vi "Sorted ARR Data.vi"(10 "Uart-num":string[](array[string])=["11", "15"], 11 "Data":string[][](array[string])=[["0", "11", "12"], ["15", "11", "11"], ["11", "11", "11"], ["12", "11", "11"], ["15", "11", "11"]]) -> (2 "Consistent":bool, 3 "Data-Sorted":string[][](array[string]))   [LabVIEW 2025, in "G-Uart-Class.lvclass"]
uses:
  G-Uart-Class.lvclass
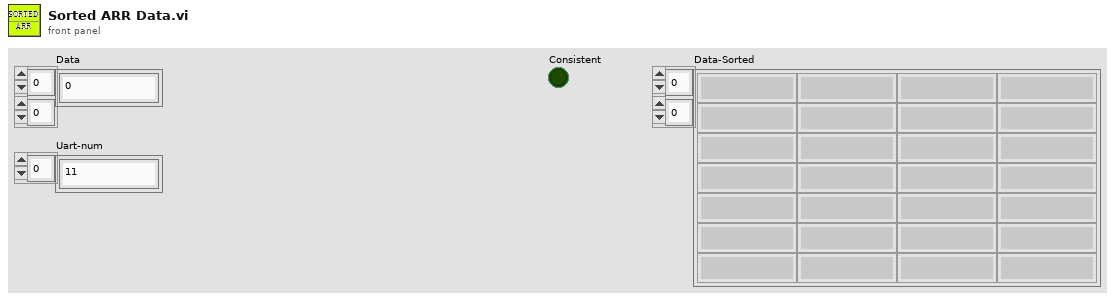
[diagram p1: front panel]
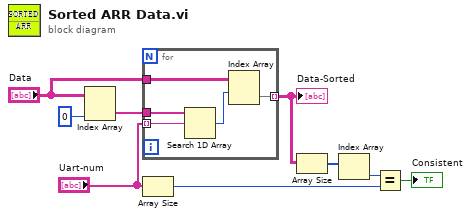
[diagram p0: block diagram]
diagram:
  n1 = Index Array(array="Data", index (col)=0 ("禁用的索引 (列)")) -> (element=w8:string[])  [unwired: 1 in]
  n2 = for {
    tunnel: w8 -> [w13]
    tunnel: "Uart-num" -> [w14] mode=indexing
    tunnel: "Data" -> [w12]
    tunnel: [w10] -> w1 mode=indexing
    n3 = Search 1D Array(1D array=w13, element=w14) -> (index of element=w11:i32)  [unwired: 1 in]
    n4 = Index Array(array=w12, index (row)=w11) -> (element=w10:string[])  [unwired: 1 in]
  }
  "Data-Sorted" <- w1
  n5 = Array Size(array="Uart-num") -> (size(s)=w4:i32)
  n6 = Array Size(array=w1) -> (size(s)=w6:i32[])
  n7 = Index Array(array=w6) -> (element=w5:i32)  [unwired: 1 in]
  n8 = Equal?(x=w5, y=w4) -> (x = y?=→"Consistent":bool)
